vi "AdaptToInputs.vi"(3 "Term Types":T1[](array[typedef]), 4 "XRef":refnum<vi>, 5 "State In":T4) -> (0 "Reply":string[](array[string]), 2 "State Out":T4)   [LabVIEW 2012, in "Unindex and Unbundle.xnode"]
doc: "This ability VI is called by LabVIEW during type propagation so that your XNode may adapt itself to new input types. Term Types is an array of pairs of current Term IDs and the type descriptors corresponding to them. The type descriptors are taken from the signal connected to the terminal. Unwired terminals are not included in the array. Use Reply to inform LabVIEW of any actions it needs to take.\n\nDefault behavior: None.\n\nThis ability does not provide UI and OS messages are not handled."
uses:
  Unindex and Unbundle.xnode
  State.ctl
  <vilib>/XNodeSupport/XNodeTermTypeIDPair.ctl
  <vilib>/XNodeSupport/XNodeType.ctl
  <vilib>/XNodeSupport/XNodeString.ctl
  <vilib>/Utility/VariantDataType/VariantType.lvlib
  <vilib>/XNodeSupport/NI_XNodeSupport.lvlib
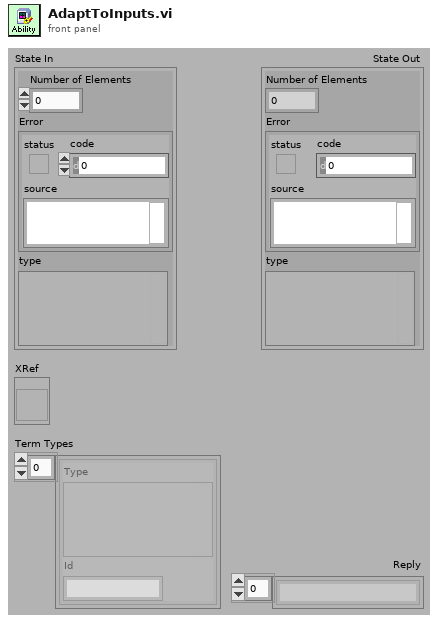
[diagram p1: front panel]
types:
  T1 = typedef "NI_XNodeSupport.lvlib/XNodeTermTypeIDPair.ctl" = cluster{"Type":T2, "Id":T3}
  T2 = typedef "NI_XNodeSupport.lvlib/XNodeType.ctl" = variant
  T3 = typedef "NI_XNodeSupport.lvlib/XNodeString.ctl" = string
  T4 = typedef "Unindex and Unbundle.xnode/State.ctl" = cluster{"Number of Elements":i32, "Error":errorcluster, "type":variant}
  T5 = typedef "VariantType.lvlib/Type.ctl" = enum8{"Invalid Type", "Void", "I8", "I16", "I32", "I64", "U8", "U16", "U32", "U64", "Single Float", "Double Float", "Extended Float", "Single Complex", "Double Complex", "Extended Complex", "Enum U8", "Enum U16", "Enum U32", "Enum U64", "Single Float With Unit", "Double Float With Unit", "Extended Float With Unit", "Single Complex with Unit", "Double Complex with Unit", "Extended Complex with Unit", "Boolean", "String", "Path", "Picture", "Tag", "Array", "Cluster", "Variant", "LV Variant", "Waveform", "Timestamp", "Digital Waveform", "Digital Data", "ExpressData", "Refnum", "External Data", "VI", "Poly VI", "LabVIEW Class Instance", "Fixed Point"}
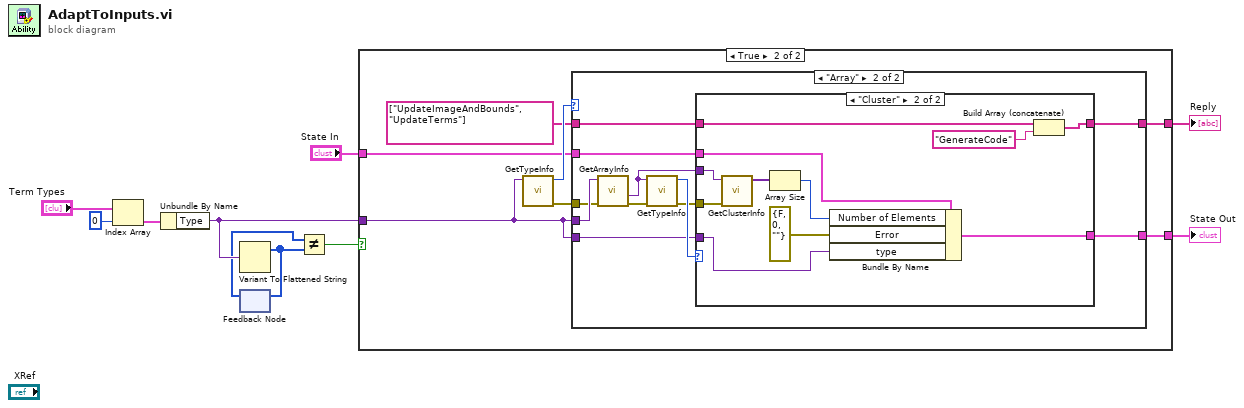
[diagram p0: block diagram]
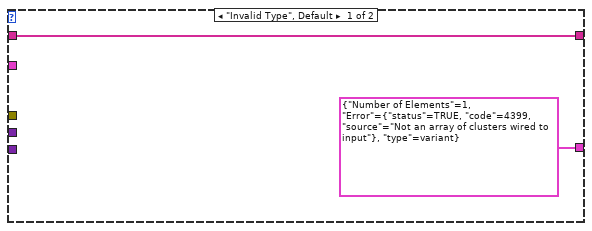
[diagram p3: hidden frame]
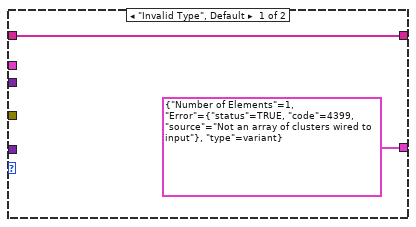
[diagram p4: hidden frame]
diagram:
  n1 = Index Array(array="Term Types", index=0) -> (element=w8:T1)
  n2 = Unbundle By Name(w8) -> ("Type"=w5:T2)
  n3 = Variant To Flattened String(Variant=w5) -> (1:w3:i16[])  [unwired: 1 out]
  n4 = feedback-in #1(w3) -> ()
  n5 = feedback #1() -> (w4:i16[])  [unwired: 1 out]
  n6 = Not Equal?(x=w4, y=w3) -> (x != y?=w1:bool)
  n7 = case shown="True" w1 {
    tunnel: "State In" -> [w11 w17]
    tunnel: [w11 w16] -> w6
    tunnel: w5 -> [_ w13]
    tunnel: [_ w12] -> w2
    frame False {
    }
    frame True {
      n8 = call <vilib>:"GetTypeInfo.vi"("Variant"=w13) -> ("error out"=w14:errorcluster, "Type Enum"=w18:T5)  [unwired: 1 in, 8 out]
      n9 = case shown="\"Array\"" w18 {
        tunnel: w13 -> [_ w31]
        tunnel: w17 -> [_ w28]
        tunnel: [T4 {"Number of Elements"=1, "Error"={"status"=TRUE, "code"=4399, "source"="Not an array of clusters wired to input"}, "type"=variant} ("State In") w26] -> w16
        tunnel: [w19 w25] -> w12
        tunnel: string[] ["UpdateImageAndBounds", "UpdateTerms"] ("Reply") -> [w19 w24]
        tunnel: w14 -> [_ w23]
        tunnel: w13 -> [_ w21]
        frame "Invalid Type", Default {
        }
        frame "Array" {
          n10 = call <vilib>:"GetArrayInfo.vi"("error in (no error)"=w23, "Variant"=w31) -> ("error out"=w30:errorcluster, "ArrayElement"=w27:variant)  [unwired: 8 out]
          n11 = call <vilib>:"GetTypeInfo.vi"("error in (no error)"=w30, "Variant"=w27) -> ("error out"=w22:errorcluster, "Type Enum"=w29:T5)  [unwired: 8 out]
          n12 = case shown="\"Cluster\"" w29 {
            tunnel: w28 -> [_ w44]
            tunnel: w27 -> [_ w43]
            tunnel: [T4 {"Number of Elements"=1, "Error"={"status"=TRUE, "code"=4399, "source"="Not an array of clusters wired to input"}, "type"=variant} ("State In") w39] -> w26
            tunnel: [w32 w37] -> w25
            tunnel: w24 -> [w32 w38]
            tunnel: w22 -> [_ w35]
            tunnel: w21 -> [_ w34]
            frame "Invalid Type", Default {
            }
            frame "Cluster" {
              n13 = call <vilib>:"GetClusterInfo.vi"("error in (no error)"=w35, "Variant"=w43) -> ("Cluster Elements"=w42:variant[])  [unwired: 9 out]
              n14 = Array Size(array=w42) -> (size(s)=w41:i32)
              n15 = Bundle By Name(cluster=w44, "Number of Elements"=w41, "Error"=errorcluster {"status"=FALSE, "code"=0, "source"=""}, "type"=w34) -> (w39:T4)
              n16 = Build Array (concatenate)(w38, "GenerateCode") -> (w37:string[])
            }
          }
        }
      }
    }
  }
  "Reply" <- w2
  "State Out" <- w6
